vi "ask_data_core.vi"(0 "agent_simple_qa in":refnum<class "agent_simple_qa.lvclass">, 5 "message":refnum<class "abstract_message_base.lvclass">, 11 "error in (no error)":errorcluster) -> (4 "agent_simple_qa out":refnum<class "agent_simple_qa.lvclass">, 6 "assisstant_response":refnum<class "abstract_message_base.lvclass">, 15 "error out":errorcluster)   [LabVIEW 2020, in "agent_simple_qa.lvclass"]
uses:
  agent_simple_qa.lvclass
  models/abstract_message_base/abstract_message_base.lvclass
  agent_simple_qa.lvclass/agent_simple_qa.ctl
  models/message_text/message_text.lvclass
  D:/Personal/LabVIEW LLMs/src/models/abstract_message_base/abstract_message_base.lvclass
  models/message_vectors/message_vectors.lvclass
  models/message_vectors/get_vector_message_value.vi
  vectorstore/abstract_vector_base/abstract_vector_base.lvclass
  models/abstract_llm_chatcompletion/abstract_llm_chatcompletion.lvclass
  models/abstract_llm_embedding/abstract_llm_embedding.lvclass
  D:/Personal/LabVIEW LLMs/src/models/message_vectors/message_vectors.lvclass
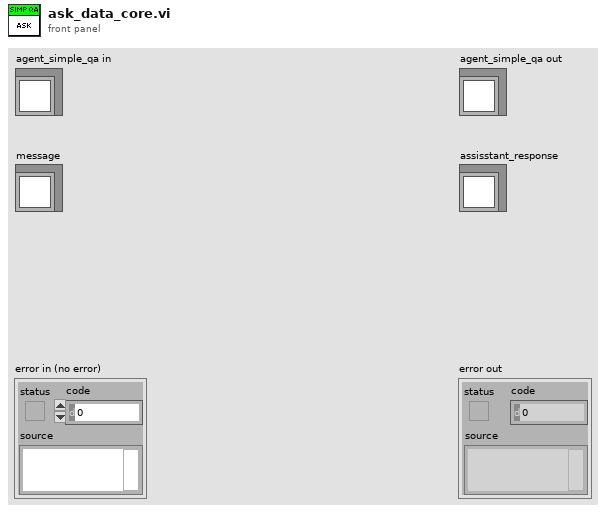
[diagram p1: front panel]
types:
  T1 = typedef "message_vectors.lvclass/embedding.ctl" = cluster{"index":u32, "Vectors":dbl[]}
  T2 = typedef "abstract_vector_base.lvclass/search result.ctl" = cluster{"score":dbl, "vector":T3}
  T3 = typedef "abstract_vector_base.lvclass/vector.ctl" = cluster{"id":string, "vector":dbl[], "text":string, "metadata":cluster{"key":string, "value":string}[]}
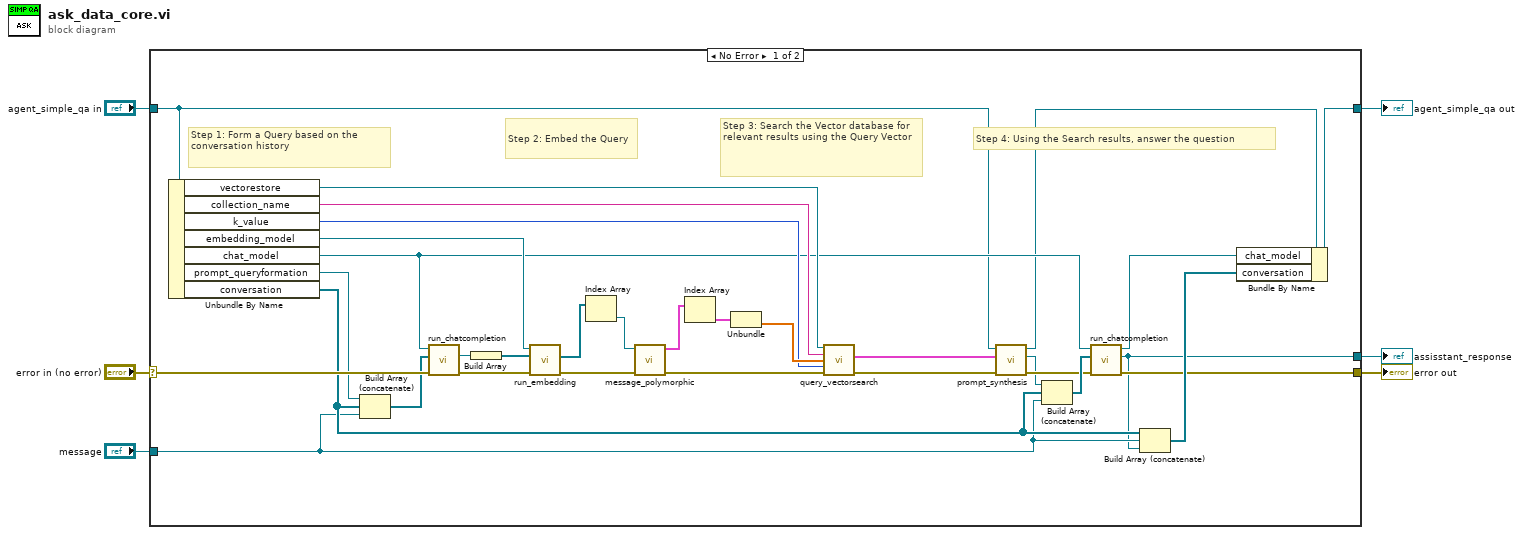
[diagram p0: block diagram]
diagram:
  n1 = case shown="No Error" "error in (no error)" {
    selector: "error in (no error)" -> [w34 w40]
    tunnel: [w8 w40] -> w5
    tunnel: [w37 w39] -> w3
    tunnel: "agent_simple_qa in" -> [w14 w39]
    tunnel: "message" -> [w9 _]
    tunnel: [w7 _] -> w2
    frame No Error {
      # "Step 4: Using the Search results, answer the question"
      # "Step 2: Embed the Query"
      # "Step 3: Search the Vector database for relevant results using the Query Vector"
      # "Step 1: Form a Query based on the conversation history"
      n2 = Unbundle By Name(w14) -> ("vectorestore"=w31:refnum<class "abstract_vector_base.lvclass">, "collection_name"=w30:string, "k_value"=w18:u32, "embedding_model"=w29:refnum<class "abstract_llm_base.lvclass">, "chat_model"=w17:refnum<class "abstract_llm_base.lvclass">, "prompt_queryformation"=w32:refnum<class "message_text.lvclass">, "conversation"=w10:refnum<class "abstract_message_base.lvclass">[])
      n3 = Build Array (concatenate)(w32, w10, w9) -> (w33:refnum<class "abstract_message_base.lvclass">[])
      n4 = call "run_chatcompletion.vi"("error in (no error)"=w34, "Messages"=w33, "abstract_llm_chatcompletion in"=w17) -> ("error out"=w28:errorcluster, "Response"=w27:refnum<class "abstract_message_base.lvclass">)  [unwired: 6 in, 1 out]
      n5 = Build Array(w27) -> (w26:refnum<class "abstract_message_base.lvclass">[])
      n6 = call "run_embedding.vi"("error in (no error)"=w28, "Messages"=w26, "abstract_llm_embedding in"=w29) -> ("error out"=w23:errorcluster, "Response"=w25:refnum<class "message_vectors.lvclass">[])  [unwired: 6 in, 1 out]
      n7 = Index Array(array=w25) -> (element=w24:refnum<class "message_vectors.lvclass">)  [unwired: 1 in]
      n8 = call-poly "message_polymorphic.vi"("error in (no error)"=w23, "message_vectors in"=w24) -> ("error out"=w19:errorcluster, "embedding_data"=w22:T1[])  [unwired: 8 in]
      n9 = Index Array(array=w22) -> (element=w21:T1)  [unwired: 1 in]
      n10 = Unbundle(w21) -> ("Vectors"=w20:dbl[])  [unwired: 1 out]
      n11 = call-dynamic "query_vectorsearch.vi"("abstract_vector_base in"=w31, "collection_name"=w30, "vector"=w20, "limit"=w18, "error in (no error)"=w19) -> ("results"=w12:T2[], "error out"=w16:errorcluster)  [unwired: 8 in, 1 out]
      n12 = call "prompt_synthesis.vi"("error in (no error)"=w16, "search_results"=w12, "agent_simple_qa in"=w14) -> ("error out"=w15:errorcluster, "prompt_synthesiser"=w11:refnum<class "message_text.lvclass">, "agent_simple_qa out"=w13:refnum<class "agent_simple_qa.lvclass">)  [unwired: 6 in]
      n13 = Build Array (concatenate)(w11, w10, w9) -> (w36:refnum<class "abstract_message_base.lvclass">[])
      n14 = call "run_chatcompletion.vi"("error in (no error)"=w15, "Messages"=w36, "abstract_llm_chatcompletion in"=w17) -> ("error out"=w8:errorcluster, "Response"=w7:refnum<class "abstract_message_base.lvclass">, "abstract_llm_chatcompletion out"=w38:refnum<class "abstract_llm_base.lvclass">)  [unwired: 6 in]
      n15 = Build Array (concatenate)(w10, w9, w7) -> (w35:refnum<class "abstract_message_base.lvclass">[])
      n16 = Bundle By Name(cluster=w13, "chat_model"=w38, "conversation"=w35) -> (w37:refnum<class "agent_simple_qa.lvclass">)
    }
    frame Error {
    }
  }
  "error out" <- w5
  "agent_simple_qa out" <- w3
  "assisstant_response" <- w2
